vi "VIPM Post Uninstall Process.vi"(7 "vi.lib relative path (Viviota\\shared)":path=path "Viviota/shared", 8 "Error In":errorcluster, 11 "PackageName":string) -> (0 "Error Out":errorcluster)   [LabVIEW 2020]
uses:
  <vilib>/Utility/file.llb/Read Delimited Spreadsheet (string).vi
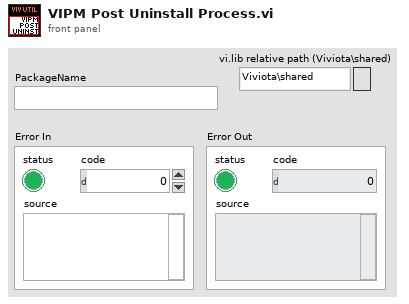
[diagram p1: front panel]
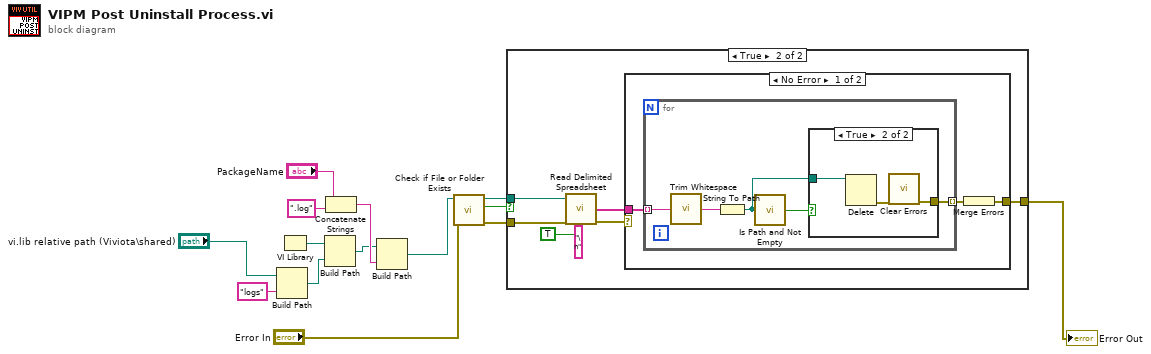
[diagram p0: block diagram]
diagram:
  n1 = Build Path(base path="vi.lib relative path (Viviota\\shared)", name or relative path="logs") -> (appended path=w2:path)
  n2 = VI Library() -> (path=w8:path)
  n3 = Build Path(base path=w8, name or relative path=w2) -> (appended path=w7:path)
  n4 = Concatenate Strings("PackageName", ".log" ("string")) -> (w13:string)
  n5 = Build Path(base path=w7, name or relative path=w13) -> (appended path=w9:path)
  n6 = call <vilib>:"Check if File or Folder Exists.vi"("error in (no error)"="Error In", "path"=w9) -> ("error out"=w10:errorcluster, "file or folder exists?"=w12:bool, "dup path"=w11:path)  [unwired: 7 in]
  n7 = case shown="True" w12 {
    tunnel: w11 -> [_ w22]
    tunnel: w10 -> [w15 w19]
    tunnel: [w15 w16] -> w4
    frame False {
    }
    frame True {
      n8 = call-poly <vilib>:"Read Delimited Spreadsheet.vi"("file path (dialog if empty)"=w22, "error in (no error)"=w19, "transpose? (F)"=TRUE, "delimiter (\\t)"="\n" ("delimiter (\\t)")) -> ("first row"=w20:string[], "error out"=w18:errorcluster)  [unwired: 6 in, 4 out]
      n9 = case shown="No Error" w18 {
        selector: w18 -> [_ w34]
        tunnel: w20 -> [w25 _]
        tunnel: [w23 w34] -> w16
        frame No Error {
          n10 = for {
            tunnel: w25 -> [w30] mode=indexing
            tunnel: [w26] -> w24 mode=indexing
            n11 = call <vilib>:"Trim Whitespace.vi"("string"=w30) -> ("trimmed string"=w29:string)  [unwired: 1 in]
            n12 = String To Path(string=w29) -> (path=w27:path)
            n13 = call <vilib>:"Is Path and Not Empty.vi"("path"=w27) -> ("Is Path and Not Empty?"=w28:bool)  [unwired: 4 in]
            n14 = case shown="True" w28 {
              tunnel: w27 -> [_ w33]
              tunnel: [_ w31] -> w26
              frame False {
              }
              frame True {
                n15 = Delete(path (use dialog)=w33) -> (error out=w32:errorcluster)  [unwired: 4 in, 2 out]
                n16 = call <vilib>:"Clear Errors.vi"("error in (no error)"=w32) -> ("error out"=w31:errorcluster)  [unwired: 5 in, 1 out]
              }
            }
          }
          n17 = Merge Errors(w24) -> (w23:errorcluster)
        }
        frame Error {
        }
      }
    }
  }
  "Error Out" <- w4
